vi "user32 GetCursorPos.vi"(11 "error in":errorcluster) -> (4 "X":i32, 6 "Y":i32, 8 "return value":i32, 15 "error out":errorcluster)   [LabVIEW 2020, in "RemoteVI.lvlib"]
doc: "Reads the mouse cursor position in SCREEN coordinates through user32.dll GetCursorPos (stdcall, called in any thread). The point travels to the DLL as a POINT {LONG x, LONG y} that the function overwrites in place. return value is the Win32 BOOL: non-zero on success, 0 on failure. When error in carries an error the DLL is not called. Generated by scripts\\Build Win32 Wrappers.vi - do not edit by hand, rebuild it."
uses:
  RemoteVI.lvlib
  user32.dll
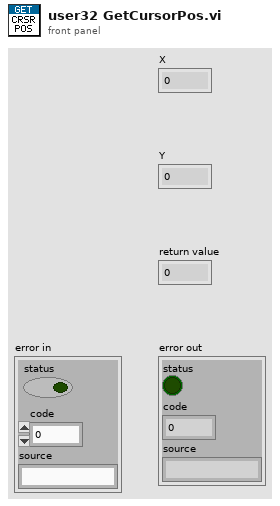
[diagram p1: front panel]
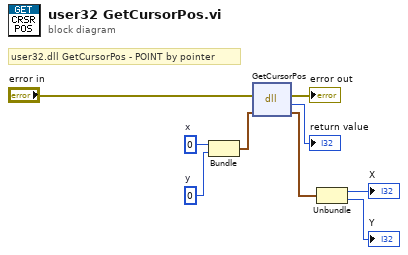
[diagram p0: block diagram]
diagram:
  w9 = 0  # y
  w8 = 0  # x
  # "user32.dll GetCursorPos - POINT by pointer"
  n1 = Bundle("x"=w8, "y"=w9) -> (w2:cluster{"x":i32, "y":i32})  [unwired: 1 in]
  n2 = dll-call lib="user32.dll" fn="GetCursorPos"(error in="error in", "lpPoint"=w2) -> (error out=→"error out":errorcluster, →"return value":i32, "lpPoint"=w1:cluster{"x":i32, "y":i32})  [unwired: 2 in, 1 out]
  n3 = Unbundle(w1) -> ("x"=→"X":i32, "y"=→"Y":i32)
